vi "VIH Utility - FILE - Get Top-Level VI Path & Directory.vi"(8 "error in":errorcluster) -> (0 "error out":errorcluster, 1 "VI Directory out of .LLB":path, 2 "VI Directory Path":path, 3 "VI Path":path)   [LabVIEW 2014]
doc: "::: VI Helpeks :::\nCopyright (c) 2000-2026 Konstantin Shifershteyn. All rights reserved."
panel:
  # "VI Helpeks\nCopyright (c) 2012-2026 Konstantin Shifershteyn"
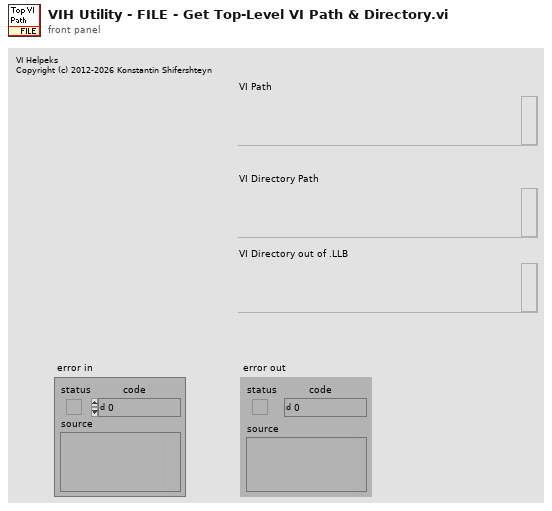
[diagram p1: front panel]
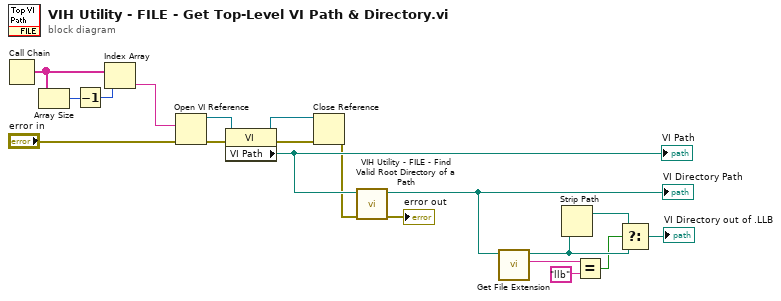
[diagram p0: block diagram]
diagram:
  n1 = Call Chain() -> (call chain=w11:string[])
  n2 = Array Size(array=w11) -> (size(s)=w12:i32)
  n3 = Decrement(x=w12) -> (x-1=w13:i32)
  n4 = Index Array(array=w11, index=w13) -> (element=w14:string)
  n5 = Open VI Reference(vi path=w14, error in (no error)="error in") -> (vi reference=w10:refnum<vi>, error out=w9:errorcluster)  [unwired: 4 out]
  n6 = property class="VI"(reference=w10, error in=w9) -> (reference out=w18:refnum<vi>, error out=w19:errorcluster, "VI Path"=w17:path)
  "VI Path" <- w17
  n7 = Close Reference(reference=w18, error in (no error)=w19) -> (error out=w16:errorcluster)
  n8 = call "VIH Utility - FILE - Find Valid Root Directory of a Path.vi"("error in"=w16, "Path in"=w17) -> ("error out"=→"error out":errorcluster, "Root directory path"=w2:path)  [unwired: 7 in, 1 out]
  "VI Directory Path" <- w2
  n9 = call <vilib>:"Get File Extension.vi"("file"=w2) -> ("lowercase file extension"=w4:string, "dup file"=w6:path)  [unwired: 7 in, 2 out]
  n10 = Strip Path(path=w6) -> (stripped path=w7:path)  [unwired: 1 out]
  n11 = Equal?(x=w4, y="llb" ("x")) -> (x = y?=w3:bool)
  n12 = Select(t=w7, s=w3, f=w6) -> (s? t:f=→"VI Directory out of .LLB":path)
